vi "Check Replacement Map.vi"(10 "Replace Column":T1, 11 "Replace Map":map{T1, u16}(c390)) -> (1 "Replace Value":u16, 3 "Replace Map out":map{T1, u16}(c390))   [LabVIEW 2020, in "VI Properties Editor.lvlib"]
doc: "Checks <B>Replace Map</B> for the last <B>Replace Value</B> used with <B>Replace Column</B>."
uses:
  VI Properties Editor.lvlib
  CTLs/Replace Column.ctl
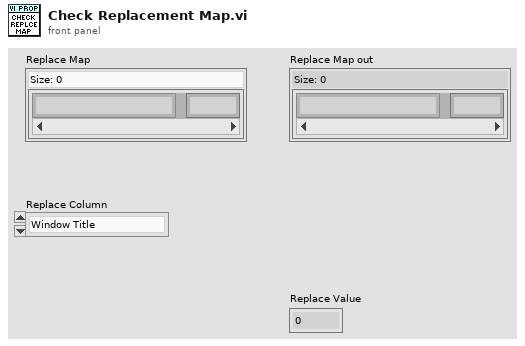
[diagram p1: front panel]
types:
  T1 = typedef "VI Properties Editor.lvlib/Replace Column.ctl" = enum16{"Window Title", "Description", "Help Path", "Help Tag", "Custom Title?", "Help URL", "Help Type", "Inlined?", "Allow debugging?", "Auto error handling?", "Run when opened?", "Suspend when called?", "Reentrancy", "Priority", "Preferred Exec System", "Control Label", "Control Caption", "Control Description", "Control Tip Strip"}
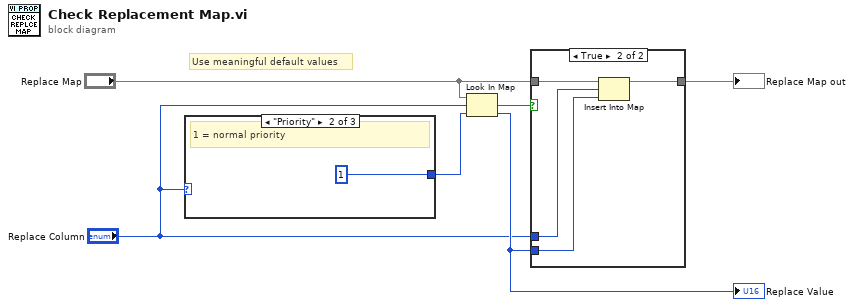
[diagram p0: block diagram]
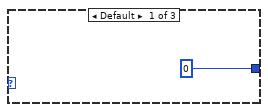
[diagram p2: hidden frame]
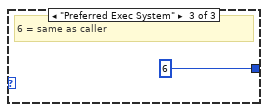
[diagram p3: hidden frame]
diagram:
  # "Use meaningful default values"
  n1 = case shown="\"Priority\"" "Replace Column" {
    tunnel: [u16 0 u16 1 u16 6] -> w1
    frame Default {
    }
    frame "Priority" {
      # "1 = normal priority"
    }
    frame "Preferred Exec System" {
      # "6 = same as caller"
    }
  }
  n2 = Look In Map(map="Replace Map", key="Replace Column", default value=w1) -> (key not found?=w6:bool, value=w3:u16)
  "Replace Value" <- w3
  n3 = case shown="True" w6 {
    tunnel: w3 -> [_ w12]
    tunnel: "Replace Map" -> [w10 w14]
    tunnel: [w10 w13] -> w4
    tunnel: "Replace Column" -> [_ w11]
    frame False {
    }
    frame True {
      n4 = Insert Into Map(map in=w14, key=w11, value=w12) -> (map out=w13:map{T1, u16})  [unwired: 2 out]
    }
  }
  "Replace Map out" <- w4
